vi "Get All Test Events.vi"(8 "error in (no error)":errorcluster, 11 "Test Event Storage in":refnum<class "Test Event Storage.lvclass">) -> (0 "error out":errorcluster, 2 "Test IDs":string[](array[string]), 3 "Test Event Storage out":refnum<class "Test Event Storage.lvclass">, 4 "Assertions":T1[](array[typedef]))   [LabVIEW 2020, in "Caraya.lvlib" / "Test Event Storage.lvclass"]
uses:
  Test Event Storage.lvclass
  Test Result/Assert Event Data (Extended).ctl
  assert store -- cluster.ctl
  Test Manager Message Assertion/TestManagerMsg.Assertion.lvclass
  C:/projects/caraya/src/classes/Test Manager Message/TestManagerMsg.lvclass
  Test Manager Message Verbose/TestManagerMsg.Verbose.lvclass
  Test Event Storage.lvclass/Test Event Storage.ctl
  Test Manager Message/TestManagerMsg.lvclass/TestManagerMsg.ctl
  Test Manager Message/TestManagerMsg.lvclass
  Test Result/Test Result.lvclass
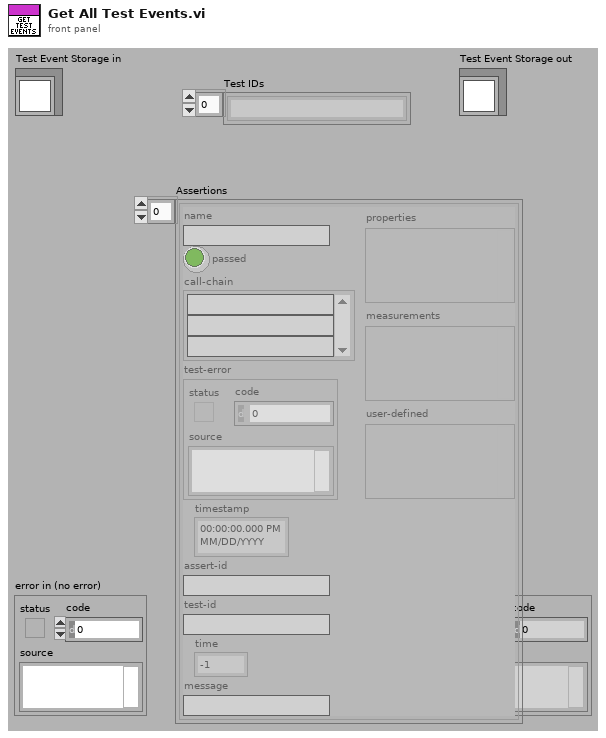
[diagram p1: front panel]
types:
  T1 = typedef "Caraya.lvlib/Test Result.lvclass/Assert Event Data (Extended).ctl" = cluster{"name":string, "passed":bool, "call-chain":string[], "test-error":errorcluster, "timestamp":timestamp, "assert-id":string, "test-id":string, "time":dbl, "message":string, "properties":variant, "measurements":variant, "user-defined":variant}
  T2 = typedef "Caraya.lvlib/Test Event Storage.lvclass/assert store -- cluster.ctl" = cluster{"Assertion":refnum<class "TestManagerMsg.Assertion.lvclass">, "Explanation":refnum<class "TestManagerMsg.Verbose.lvclass">, "properties":variant, "measurements":variant, "user-defined":variant}
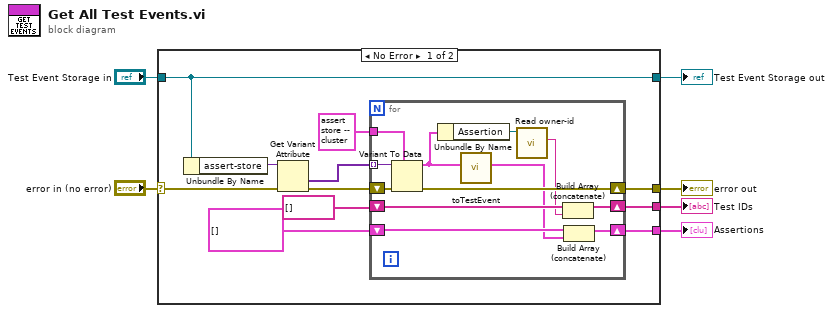
[diagram p0: block diagram]
diagram:
  n1 = case shown="No Error" "error in (no error)" {
    selector: "error in (no error)" -> [w16 w31]
    tunnel: [w17 w31] -> w5
    tunnel: [w13 w30] -> w3
    tunnel: "Test Event Storage in" -> [w13 w30]
    tunnel: [w15 _] -> w2
    tunnel: [w14 _] -> w1
    frame No Error {
      n2 = Unbundle By Name(w13) -> ("assert-store"=w12:variant)
      n3 = Get Variant Attribute(Variant=w12, error in=w16) -> (values=w11:variant[], error out=w10:errorcluster)  [unwired: 2 in, 2 out]
      n4 = for {
        tunnel: w11 -> [w29] mode=indexing
        shift-right: [w27] -> w17
        shift-left: w10 -> [w28]
        shift-right: [w26] -> w14
        shift-left: T1[] [] ("Assertions") -> [w25]
        shift-right: [w23] -> w15
        shift-left: string[] [] -> [w24]
        tunnel: T2 {"Assertion"=refnum, "Explanation"=refnum, "properties"=variant, "measurements"=variant, "user-defined"=variant} ("assert-store") -> [w22]
        n5 = Variant To Data(error in=w28, type=w22, Variant=w29) -> (data=w19:T2, error out=w27:errorcluster)
        n6 = Unbundle By Name(w19) -> ("Assertion"=w20:refnum<class "TestManagerMsg.Assertion.lvclass">)
        n7 = call "toTestEvent.vi"("assert-store"=w19) -> ("Assert Event Data"=w18:T1)  [unwired: 10 in]
        n8 = call "Read owner-id.vi"("TestManagerMsg in"=w20) -> ("owner-id"=w21:string)  [unwired: 9 in, 1 out]
        n9 = Build Array (concatenate)(w24, w21) -> (w23:string[])
        n10 = Build Array (concatenate)(w25, w18) -> (w26:T1[])
      }
    }
    frame Error {
    }
  }
  "error out" <- w5
  "Test Event Storage out" <- w3
  "Test IDs" <- w2
  "Assertions" <- w1
